vi "Ramsey_variable_tau_variable_frequency.vi"() -> ()   [LabVIEW 2024]
panel:
  out "how many ESR plots?":i32
  in  "format string":string="%f"
  in  "file (use dialog)":path
  out "output array":string[][](array[string])
  in  "How many passes":i32
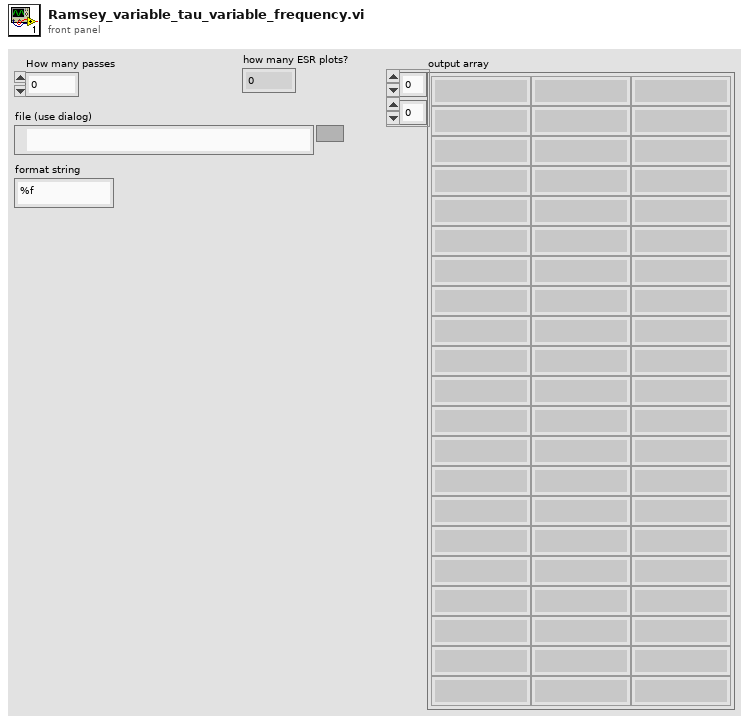
[diagram p1: front panel]
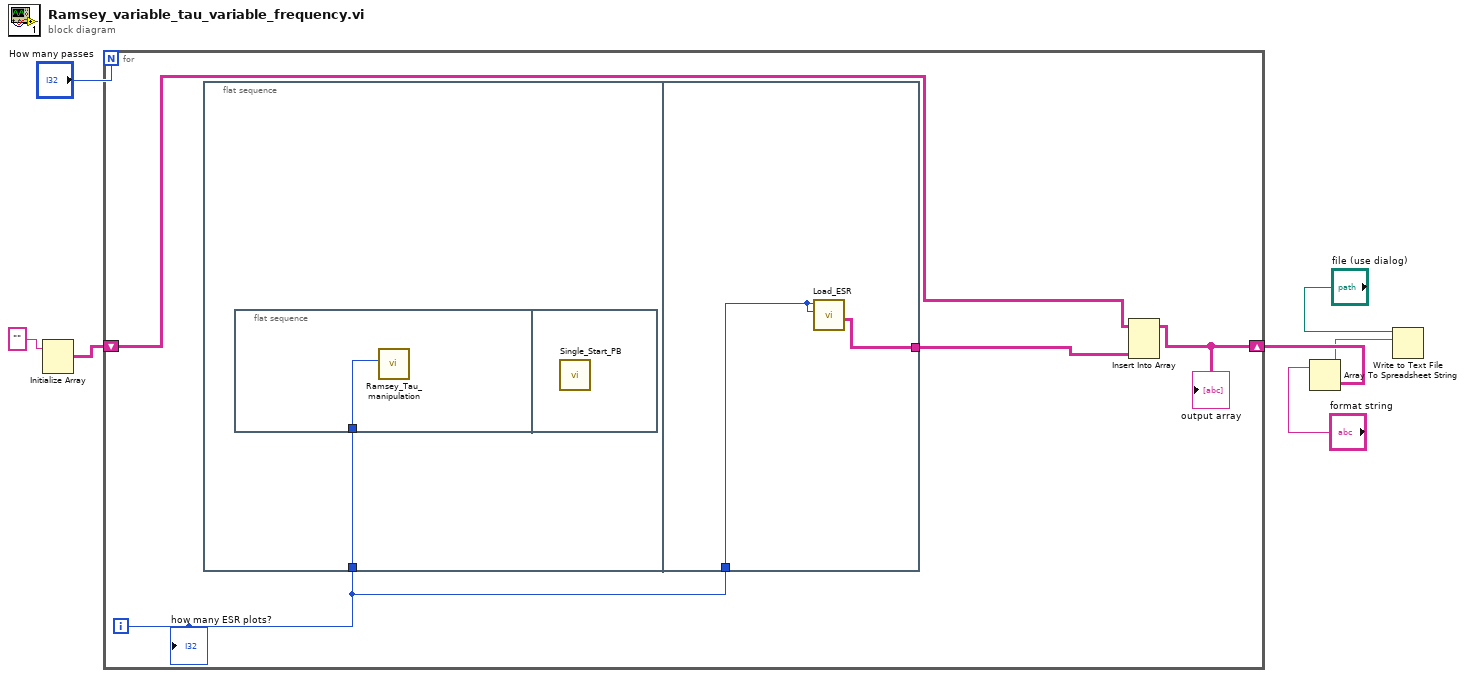
[diagram p0: block diagram]
diagram:
  n1 = Initialize Array("") -> (w6:string[][])  [unwired: 2 in]
  n2 = for {
    N: "How many passes" -> [_]
    shift-right: [w10] -> w3
    shift-left: w6 -> [w8]
    i -> [w9]
    n3 = flat-sequence {
      tunnel: w9 -> [w12]
      tunnel: [w14] -> w11
      tunnel: w9 -> [w15]
      frame #0 {
        n4 = flat-sequence {
          tunnel: w12 -> [w13]
          frame #0 {
            n5 = call "Ramsey_Tau_manipulation.vi"("Numeric"=w13) -> ()  [unwired: 10 in, 1 out]
          }
          frame #1 {
            n6 = call "Single_Start_PB.vi"() -> ()  [unwired: 12 in]
          }
        }
      }
      frame #1 {
        n7 = call "Load_ESR.vi"("wait time adjustment (inverted)"=w15, "wait time adjustment"=w15) -> ("Array"=w14:string[][])  [unwired: 7 in, 2 out]
      }
    }
    n8 = Insert Into Array(array=w8, new element=w11) -> (w10:string[][])  [unwired: 2 in]
    "output array" <- w10
    "how many ESR plots?" <- w9
  }
  n9 = Array To Spreadsheet String(array=w3, 3:"format string") -> (spreadsheet string=w2:string)  [unwired: 1 in]
  n10 = Write to Text File(file (use dialog)="file (use dialog)", text=w2) -> ()  [unwired: 2 in, 3 out]
